vi "New Reg0Write Command.vi"(0 "RFFE Reg0Write Command in":refnum<class "RFFE Reg0Write Command.lvclass">, 1 "Alias":string, 5 "Slave Address":T2=12 format="%02x", 7 "Register Data":T1 format="%02x", 11 "error in (no error)":errorcluster) -> (4 "RFFE Reg0Write Command out":refnum<class "RFFE Reg0Write Command.lvclass">, 15 "error out":errorcluster)   [LabVIEW 2018, in "MIPI RFFE API.lvlib" / "RFFE Reg0Write Command.lvclass"]
uses:
  RFFE Reg0Write Command.lvclass
  C:/Users/semoore/Projects/mipi-rffe-labview-oop/Command/RFFE Command.lvclass
  Slave Address.ctl
  Register Data.ctl
  Register Address.ctl
  RFFE Reg0Write Command.lvclass/RFFE Reg0Write Command.ctl
  Command/RFFE Command.lvclass
  MIPI RFFE API.lvlib
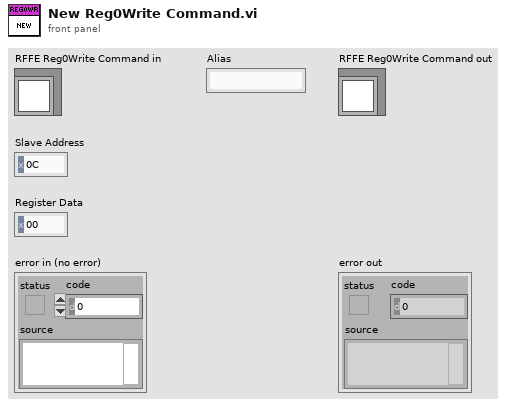
[diagram p1: front panel]
types:
  T1 = typedef "MIPI RFFE API.lvlib/Register Data.ctl" = u8
  T2 = typedef "MIPI RFFE API.lvlib/Slave Address.ctl" = u8
  T3 = typedef "MIPI RFFE API.lvlib/Register Address.ctl" = u16
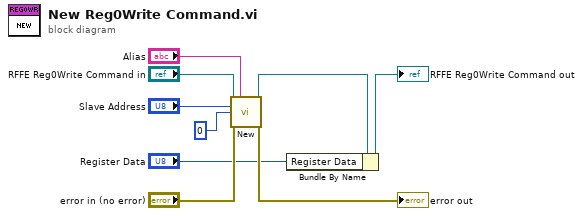
[diagram p0: block diagram]
diagram:
  n1 = call "New.vi"("RFFE Command in"="RFFE Reg0Write Command in", "Alias"="Alias", "Slave Address"="Slave Address", "Register Address"=T3 0, "error in (no error)"="error in (no error)") -> ("RFFE Command out"=w3:refnum<class "RFFE Reg0Write Command.lvclass">, "error out"=→"error out":errorcluster)  [unwired: 9 in]
  n2 = Bundle By Name(cluster=w3, "Register Data"="Register Data") -> (→"RFFE Reg0Write Command out":refnum<class "RFFE Reg0Write Command.lvclass">)
